vi "Configuration Parse.vi"(8 "error in":errorcluster, 11 "Measurement Configuration":T6={"Automation Test"=FALSE, "Power sequencing file path"="", "RFSG name"="5842", "RFSG port"="port1", "RFSG attenuation mode"=enum."<None>", "RFSG external attenuation (dB)"=2.0, "RFSG s-parameters orientation"=enum."Port1 Towards DUT", "RFSG s2p file path"="", "RFmx name"="5842", "RFmx port"="port2", "RFmx attenuation mode"=enum."<None>", "RFmx external attenuation (dB)"=11.2, "RFmx s-parameters orientation"=enum."Port1 Towards DUT", "RFmx s2p file path"="", "RFmx Reference Level (dBm)"=20.0, "RFSG Generation IQ Rate (S/s)"=30000000.0, "Target Pout Per Tone (dBm)"=0.0, "Start Pin Per Tone (dBm)"=-20.0, "Start Center Frequency (Hz)"=8000000000.0, "Start Tone Spacing (Hz)"=1000000.0, "IM_Sweep Mode"=enum."Power", "Sweep Delay (ms)"=0, "Power Sweep End"=0.0, "Power Sweep Step"=1.0, "Frequency Sweep End"=12000000000.0, "Frequency Sweep Step"=100000000.0, "Tone Spacing Sweep End"=10000000.0, "Tone Spacing Sweep Step"=1000000.0, "Power sequecing file validity check"=FALSE} {"Tone Spacing Sweep Step" format="%#.pHz"; "Tone Spacing Sweep End" format="%#.pHz"; "Frequency Sweep Step" format="%#.pHz"; "Frequency Sweep End" format="%#.pHz"; "Power Sweep Step" format="%#.fdB"; "Power Sweep End" format="%#.fdBm"; "Start Tone Spacing (Hz)" format="%#.6p"; "Start Center Frequency (Hz)" format="%#.6p"; "Start Pin Per Tone (dBm)" format="%#.6f"; "Target Pout Per Tone (dBm)" format="%#.6f"; "RFSG Generation IQ Rate (S/s)" format="%#_6p"; "RFmx Reference Level (dBm)" format="%.2f"; "RFmx external attenuation (dB)" format="%.2f"; "RFSG external attenuation (dB)" format="%.2f"}) -> (0 "error out":errorcluster, 1 "RFmx Settings":T1={"Reference Level (dBm)"=20.0, "Attenuation"={"RFmx Name"="", "RFmx Port"="", "Attenuation"={"Mode"=enum."Constant Attenuation", "Constant Attenuation"={"RFmx External Attenuation (dB)"=1.2}, "s2p File"={"RFmx S-Parameters Orientation"=24000, "RFmx Attenuation s2p Path Name"="", "RFmx Attenuation s2p File"=path ""}}}} {"Attenuation"."Attenuation"."s2p File"."RFmx S-Parameters Orientation" items=["Port1 Towards DUT"=24000, "Port2 Towards DUT"=24001]; "Attenuation"."Attenuation"."Constant Attenuation"."RFmx External Attenuation (dB)" format="%.2f"; "Reference Level (dBm)" format="%.2f"}, 2 "RFSG Settings":T3={"IQ Rate (S/sec)"=10000000.0, "Number of Samples"=3000, "Attenuation"={"RFSG Name"="5842_0", "RFSG Port"="", "Attenuation"={"Mode"=enum."Constant Attenuation", "Contant Attenuation"={"RFSG External Attenuation (dB)"=2.0}, "s2p File"={"RFSG S-parameters Orientation"=24000, "RFSG Attenuation s2p Path Name"="", "RFSG s2p File Path"=path ""}}}} {"Attenuation"."Attenuation"."s2p File"."RFSG S-parameters Orientation" items=["Port1 Towards DUT"=24000, "Port2 Towards DUT"=24001]; "Attenuation"."Attenuation"."Contant Attenuation"."RFSG External Attenuation (dB)" format="%.2f"; "IQ Rate (S/sec)" format="%#.3p"}, 3 "Test Configuration":T5={"Target Pout Per Tone (dBm)"=0.0, "Start Value"={"Power Level per Tone (dBm)"=-20.0, "Center Frequency (Hz)"=10000000000.0, "Tone Spacing (Hz)"=1000000.0}, "Sweep Settings"={"Mode"=enum."Power", "Sweep Delay (ms)"=0, "Power Sweep End"=-20.0, "Power Sweep Step"=-20.0, "Frequency Sweep End"=-4.0, "Frequency Sweep Step"=1.0, "Tone Spacing Sweep End"=-4.0, "Tone Spacing Sweep Step"=1.0}} {"Sweep Settings"."Tone Spacing Sweep Step" format="%#.pHz"; "Sweep Settings"."Tone Spacing Sweep End" format="%#.pHz"; "Sweep Settings"."Frequency Sweep Step" format="%#.pHz"; "Sweep Settings"."Frequency Sweep End" format="%#.pHz"; "Start Value"."Tone Spacing (Hz)" format="%#_6p"; "Start Value"."Center Frequency (Hz)" format="%#.3p"})   [LabVIEW 2023, in "FPT Intermodulation.lvclass"]
uses:
  FPT Intermodulation.lvclass
  Measurement Configuration.ctl
  Measurement/Controls/Test Config - TOI.ctl
  Measurement/Controls/RFSG Config - TOI.ctl
  FPT Shared VIs/De-embedding/RFsg Config.ctl
  Measurement/Controls/RFmx Config - TOI.ctl
  FPT Shared VIs/De-embedding/RFmx Config.ctl
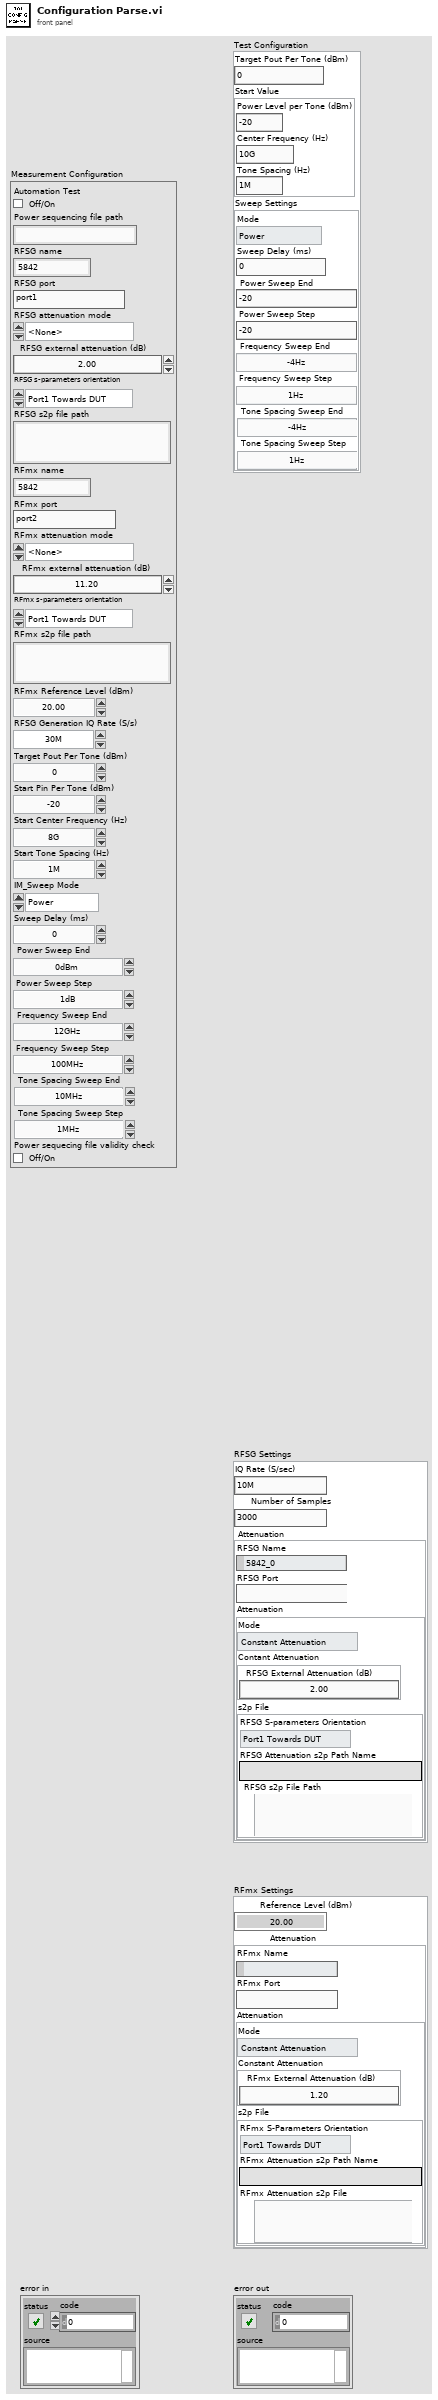
[diagram p1: front panel]
types:
  T1 = typedef "RFmx Config - TOI.ctl" = cluster{"Reference Level (dBm)":dbl, "Attenuation":T2}
  T2 = typedef "RFmx Config.ctl" = cluster{"RFmx Name":refnum<k15>, "RFmx Port":string, "Attenuation":cluster{"Mode":enum32{"<None>", "Constant Attenuation", "s2p File"}, "Constant Attenuation":cluster{"RFmx External Attenuation (dB)":dbl}, "s2p File":cluster{"RFmx S-Parameters Orientation":i32, "RFmx Attenuation s2p Path Name":string, "RFmx Attenuation s2p File":path}}}
  T3 = typedef "RFSG Config - TOI.ctl" = cluster{"IQ Rate (S/sec)":dbl, "Number of Samples":i32, "Attenuation":T4}
  T4 = typedef "RFsg Config.ctl" = cluster{"RFSG Name":refnum<k15>, "RFSG Port":string, "Attenuation":cluster{"Mode":enum32{"<None>", "Constant Attenuation", "s2p File"}, "Contant Attenuation":cluster{"RFSG External Attenuation (dB)":dbl}, "s2p File":cluster{"RFSG S-parameters Orientation":i32, "RFSG Attenuation s2p Path Name":string, "RFSG s2p File Path":path}}}
  T5 = typedef "Test Config - TOI.ctl" = cluster{"Target Pout Per Tone (dBm)":dbl, "Start Value":cluster{"Power Level per Tone (dBm)":dbl, "Center Frequency (Hz)":dbl, "Tone Spacing (Hz)":dbl}, "Sweep Settings":cluster{"Mode":enum16{"Power", "Frequency", "Tone Spacing"}, "Sweep Delay (ms)":u32, "Power Sweep End":dbl, "Power Sweep Step":dbl, "Frequency Sweep End":dbl, "Frequency Sweep Step":dbl, "Tone Spacing Sweep End":dbl, "Tone Spacing Sweep Step":dbl}}
  T6 = typedef "FPT Intermodulation.lvclass/Measurement Configuration.ctl" = cluster{"Automation Test":bool, "Power sequencing file path":string, "RFSG name":string, "RFSG port":string, "RFSG attenuation mode":enum32{"<None>", "Constant Attenuation", "s2p File"}, "RFSG external attenuation (dB)":dbl, "RFSG s-parameters orientation":enum32{"Port1 Towards DUT", "Port2 Towards DUT"}, "RFSG s2p file path":string, "RFmx name":string, "RFmx port":string, "RFmx attenuation mode":enum32{"<None>", "Constant Attenuation", "s2p File"}, "RFmx external attenuation (dB)":dbl, "RFmx s-parameters orientation":enum32{"Port1 Towards DUT", "Port2 Towards DUT"}, "RFmx s2p file path":string, "RFmx Reference Level (dBm)":dbl, "RFSG Generation IQ Rate (S/s)":dbl, "Target Pout Per Tone (dBm)":dbl, "Start Pin Per Tone (dBm)":dbl, "Start Center Frequency (Hz)":dbl, "Start Tone Spacing (Hz)":dbl, "IM_Sweep Mode":enum32{"Power", "Frequency", "Tone Spacing"}, "Sweep Delay (ms)":u32, "Power Sweep End":dbl, "Power Sweep Step":dbl, "Frequency Sweep End":dbl, "Frequency Sweep Step":dbl, "Tone Spacing Sweep End":dbl, "Tone Spacing Sweep Step":dbl, "Power sequecing file validity check":bool}
  T7 = enum32{"<None>", "Constant Attenuation", "s2p File"}
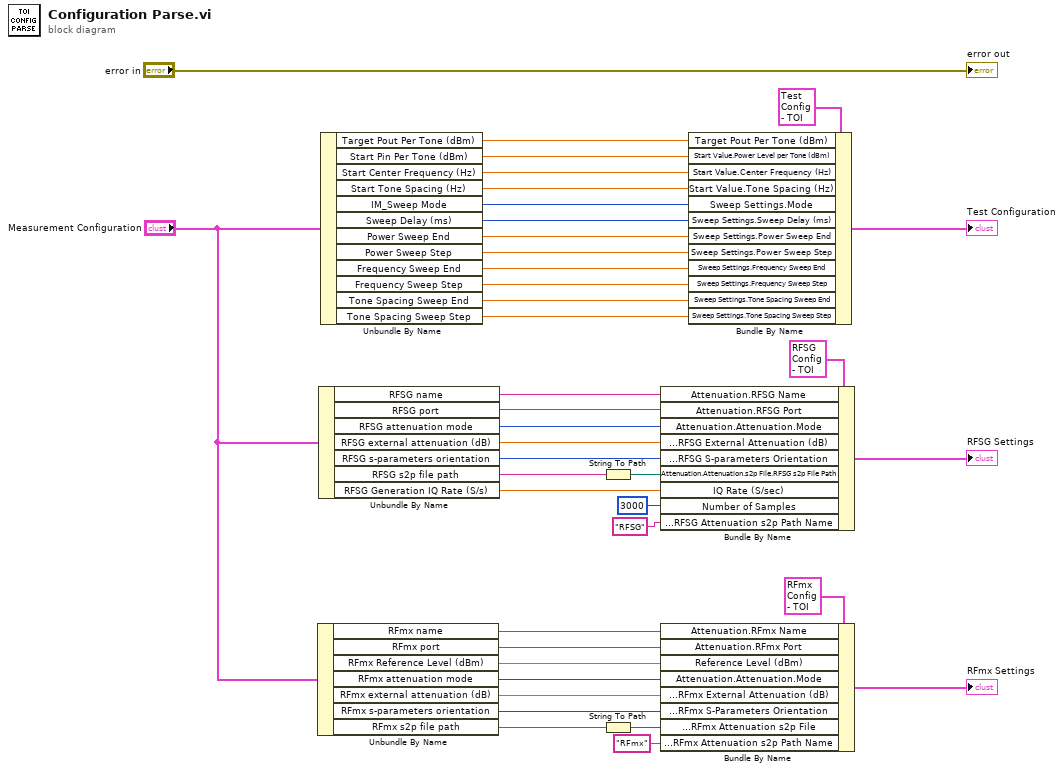
[diagram p0: block diagram]
diagram:
  n1 = Unbundle By Name("Measurement Configuration") -> ("RFmx name"=w29:string, "RFmx port"=w28:string, "RFmx Reference Level (dBm)"=w27:dbl, "RFmx attenuation mode"=w26:T7, "RFmx external attenuation (dB)"=w25:dbl, "RFmx s-parameters orientation"=w24:enum32{"Port1 Towards DUT", "Port2 Towards DUT"}, "RFmx s2p file path"=w23:string)
  n2 = Unbundle By Name("Measurement Configuration") -> ("RFSG name"=w38:string, "RFSG port"=w10:string, "RFSG attenuation mode"=w37:T7, "RFSG external attenuation (dB)"=w36:dbl, "RFSG s-parameters orientation"=w35:enum32{"Port1 Towards DUT", "Port2 Towards DUT"}, "RFSG s2p file path"=w34:string, "RFSG Generation IQ Rate (S/s)"=w20:dbl)
  n3 = Unbundle By Name("Measurement Configuration") -> ("Target Pout Per Tone (dBm)"=w18:dbl, "Start Pin Per Tone (dBm)"=w17:dbl, "Start Center Frequency (Hz)"=w16:dbl, "Start Tone Spacing (Hz)"=w15:dbl, "IM_Sweep Mode"=w14:enum32{"Power", "Frequency", "Tone Spacing"}, "Sweep Delay (ms)"=w12:u32, "Power Sweep End"=w7:dbl, "Power Sweep Step"=w6:dbl, "Frequency Sweep End"=w5:dbl, "Frequency Sweep Step"=w4:dbl, "Tone Spacing Sweep End"=w3:dbl, "Tone Spacing Sweep Step"=w2:dbl)
  n4 = String To Path(string=w34) -> (path=w33:path)
  n5 = String To Path(string=w23) -> (path=w22:path)
  n6 = Bundle By Name(cluster=T3 {"IQ Rate (S/sec)"=0.0, "Number of Samples"=0, "Attenuation"={"RFSG Name"="", "RFSG Port"="", "Attenuation"={"Mode"=enum."Constant Attenuation", "Contant Attenuation"={"RFSG External Attenuation (dB)"=0.0}, "s2p File"={"RFSG S-parameters Orientation"=24000, "RFSG Attenuation s2p Path Name"="", "RFSG s2p File Path"=path ""}}}} ("RFSG Settings"), "Attenuation.RFSG Name"=w38, "Attenuation.RFSG Port"=w10, "Attenuation.Attenuation.Mode"=w37, "Attenuation.Attenuation.Contant Attenuation.RFSG External Attenuation (dB)"=w36, "Attenuation.Attenuation.s2p File.RFSG S-parameters Orientation"=w35, "Attenuation.Attenuation.s2p File.RFSG s2p File Path"=w33, "IQ Rate (S/sec)"=w20, "Number of Samples"=3000, "Attenuation.Attenuation.s2p File.RFSG Attenuation s2p Path Name"="RFSG") -> (→"RFSG Settings":T3)
  n7 = Bundle By Name(cluster=T1 {"Reference Level (dBm)"=0.0, "Attenuation"={"RFmx Name"="", "RFmx Port"="", "Attenuation"={"Mode"=enum."Constant Attenuation", "Constant Attenuation"={"RFmx External Attenuation (dB)"=0.0}, "s2p File"={"RFmx S-Parameters Orientation"=24000, "RFmx Attenuation s2p Path Name"="", "RFmx Attenuation s2p File"=path ""}}}} ("RFmx Settings"), "Attenuation.RFmx Name"=w29, "Attenuation.RFmx Port"=w28, "Reference Level (dBm)"=w27, "Attenuation.Attenuation.Mode"=w26, "Attenuation.Attenuation.Constant Attenuation.RFmx External Attenuation (dB)"=w25, "Attenuation.Attenuation.s2p File.RFmx S-Parameters Orientation"=w24, "Attenuation.Attenuation.s2p File.RFmx Attenuation s2p File"=w22, "Attenuation.Attenuation.s2p File.RFmx Attenuation s2p Path Name"="RFmx") -> (→"RFmx Settings":T1)
  n8 = Bundle By Name(cluster=T5 {"Target Pout Per Tone (dBm)"=0.0, "Start Value"={"Power Level per Tone (dBm)"=-20.0, "Center Frequency (Hz)"=10000000000.0, "Tone Spacing (Hz)"=1000000.0}, "Sweep Settings"={"Mode"=enum."Power", "Sweep Delay (ms)"=0, "Power Sweep End"=1.0, "Power Sweep Step"=-4.0, "Frequency Sweep End"=-4.0, "Frequency Sweep Step"=1.0, "Tone Spacing Sweep End"=-4.0, "Tone Spacing Sweep Step"=1.0}} ("Test Configuration"), "Target Pout Per Tone (dBm)"=w18, "Start Value.Power Level per Tone (dBm)"=w17, "Start Value.Center Frequency (Hz)"=w16, "Start Value.Tone Spacing (Hz)"=w15, "Sweep Settings.Mode"=w14, "Sweep Settings.Sweep Delay (ms)"=w12, "Sweep Settings.Power Sweep End"=w7, "Sweep Settings.Power Sweep Step"=w6, "Sweep Settings.Frequency Sweep End"=w5, "Sweep Settings.Frequency Sweep Step"=w4, "Sweep Settings.Tone Spacing Sweep End"=w3, "Sweep Settings.Tone Spacing Sweep Step"=w2) -> (→"Test Configuration":T5)
  "error out" <- "error in"
